vi "tp_filtre_00.vi"(8 "error in (no error)":errorcluster, 10 "ID Query (True)":bool=TRUE, 11 "VISA resource name":refnum<visa-resource-name>) -> ()   [LabVIEW 2012]
doc: "Establishes communication with the instrument and optionally performs an instrument identification query and/or an instrument reset. It also places the instrument in a default state needed for other instrument driver operations. Therefore, call this VI before calling other instrument driver VIs for this instrument. Generally, you need to call the <B>Initialize VI</B> only once at the beginning of an application."
panel:
  out "decimal integer string":string
  out "concatenated string":string
  in  "Numeric":i32
  out "x = y?":bool
  # "(c) 2005-2008 National Instruments.  ALL RIGHTS RESERVED."
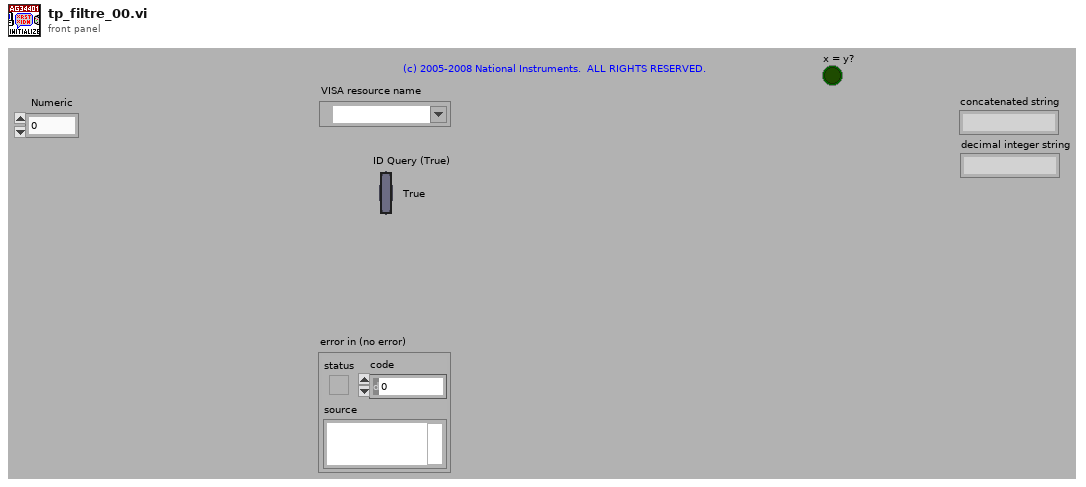
[diagram p1: front panel]
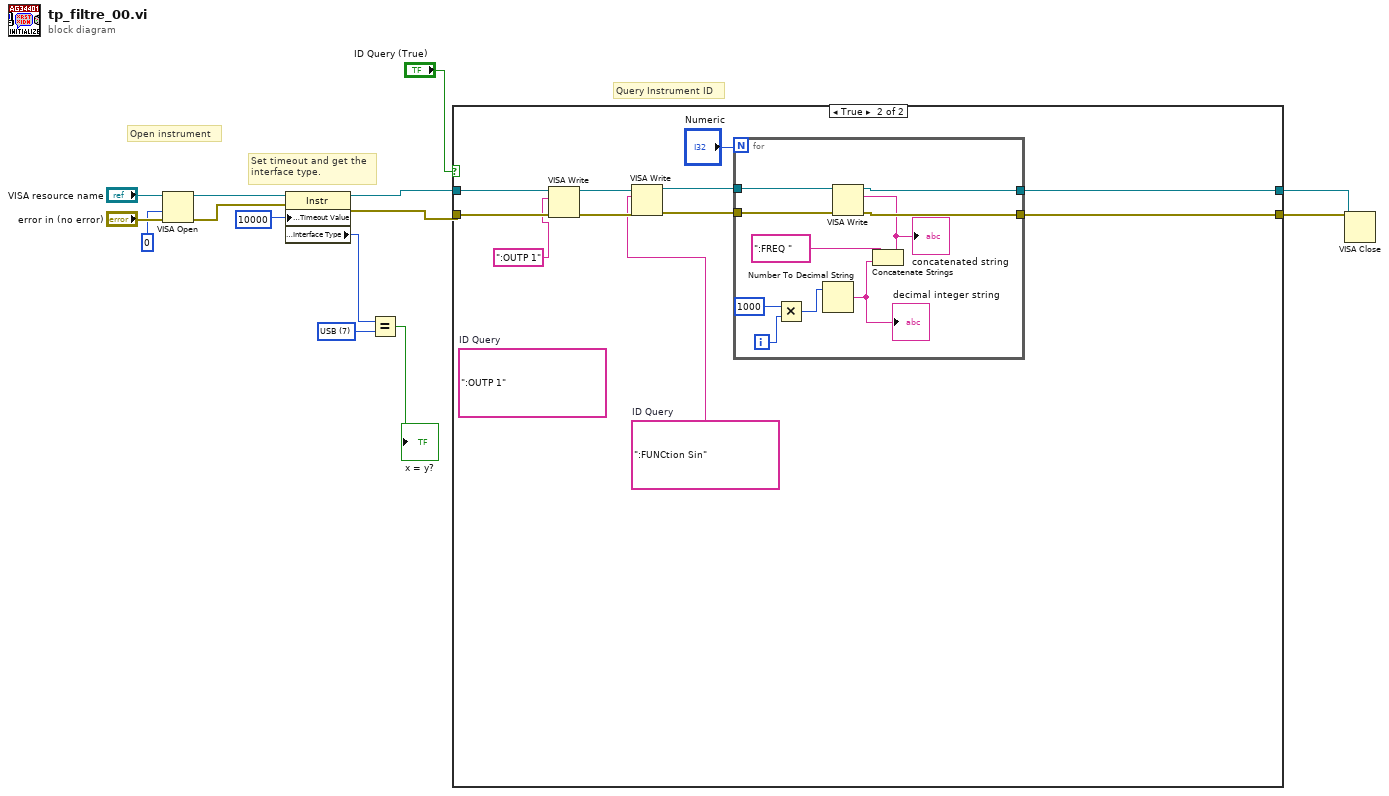
[diagram p0: block diagram]
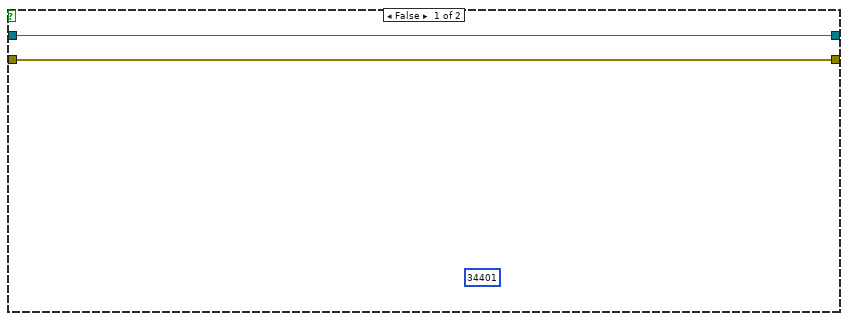
[diagram p2: hidden frame]
diagram:
  w10 = u16 7 items=["GPIB"=1, "VXI"=2, "GPIB-VXI"=3, "Serial"=4, "PXI"=5, "TCPIP"=6, "USB"=7] ("Interface Information:Interface Type")
  # "Set timeout and get the\ninterface type."
  # "Query Instrument ID"
  # "Open instrument"
  n1 = VISA Open(access mode=u32 0, error in (no error)="error in (no error)", VISA resource name="VISA resource name") -> (VISA resource name=w7:refnum<visa-resource-name>, error out=w6:errorcluster)  [unwired: 2 in]
  n2 = property on="Property Node" class="Instr"(reference=w7, error in=w6, "General Settings:Timeout Value"=u32 10000) -> (reference out=w5:refnum<visa-resource-name>, error out=w4:errorcluster, "Interface Information:Interface Type"=w12:u16)
  n3 = Equal?(x=w12, y=w10) -> (x = y?=→"x = y?":bool)
  n4 = case shown="True" "ID Query (True)" {
    tunnel: [w15 w19] -> w1
    tunnel: [w16 w20] -> w2
    tunnel: w5 -> [w16 w26]
    tunnel: w4 -> [w15 w27]
    frame False {
      (unwired) 34401
    }
    frame True {
      w23 = ":FUNCtion Sin"  # ID Query
      (unwired) ":OUTP 1"  # ID Query
      n5 = VISA Write(VISA resource name=w26, write buffer=":OUTP 1", error in (no error)=w27) -> (VISA resource name out=w25:refnum<visa-resource-name>, error out=w24:errorcluster)  [unwired: 1 out]
      n6 = VISA Write(VISA resource name=w25, write buffer=w23, error in (no error)=w24) -> (VISA resource name out=w22:refnum<visa-resource-name>, error out=w21:errorcluster)  [unwired: 1 out]
      n7 = for {
        N: "Numeric" -> [_]
        tunnel: w22 -> [w37]
        tunnel: w21 -> [w36]
        tunnel: [w34] -> w20
        tunnel: [w33] -> w19
        i -> [w29]
        n8 = Multiply(x=1000, y=w29) -> (x*y=w30:i32)
        n9 = Number To Decimal String(number=w30) -> (decimal integer string=w31:string)  [unwired: 1 in]
        "decimal integer string" <- w31
        n10 = Concatenate Strings(":FREQ ", w31) -> (w32:string)
        "concatenated string" <- w32
        n11 = VISA Write(VISA resource name=w37, write buffer=w32, error in (no error)=w36) -> (VISA resource name out=w34:refnum<visa-resource-name>, error out=w33:errorcluster)  [unwired: 1 out]
      }
    }
  }
  n12 = VISA Close(VISA resource name=w2, error in (no error)=w1) -> ()  [unwired: 1 out]
